vi "BaseProvider_ConfigurationMemory.vi"(1 "WireConfiguration":T2={"Edge thickness"=1, "Edge color"=5667411, "Center thickness"=1, "Center pattern"=enum."Solid", "CenterColor1"=9740924, "CenterColor2"=8694662, "Tunnels and terminals colors"=131187}, 2 "Icon":string="bluefull.png", 4 "Filter_Icons":bool, 5 "error in (no error)":errorcluster, 6 "Action":enum16{"Read", "Load", "Save", "Set"}(ring), 7 "PatternIn":T1 items=["4x4x4", "5x6x5", "6x8x6"]) -> (12 "ClassItemIconGroup":string[](array[string]), 13 "PatternOut":T1 items=["4x4x4", "5x6x5", "6x8x6"], 15 "WireConfigurationOut":T2={"Edge thickness"=1, "Edge color"=5667411, "Center thickness"=1, "Center pattern"=enum."Solid", "CenterColor1"=9740924, "CenterColor2"=8694662, "Tunnels and terminals colors"=131187}, 16 "IconOut":string="bluefull.png", 17 "ClassItemIconPaths":path[](array[path]), 18 "ClassItemIconNames":string[](array[string]), 19 "error out":errorcluster)   [LabVIEW 2020]
uses:
  SubVIs/GOOP_WireConfigurationType.ctl
  SubVIs/GOOP_WirePattern.ctl
  Common/ScriptingFunctions/Scripting_ConnectorPanePatternType.ctl
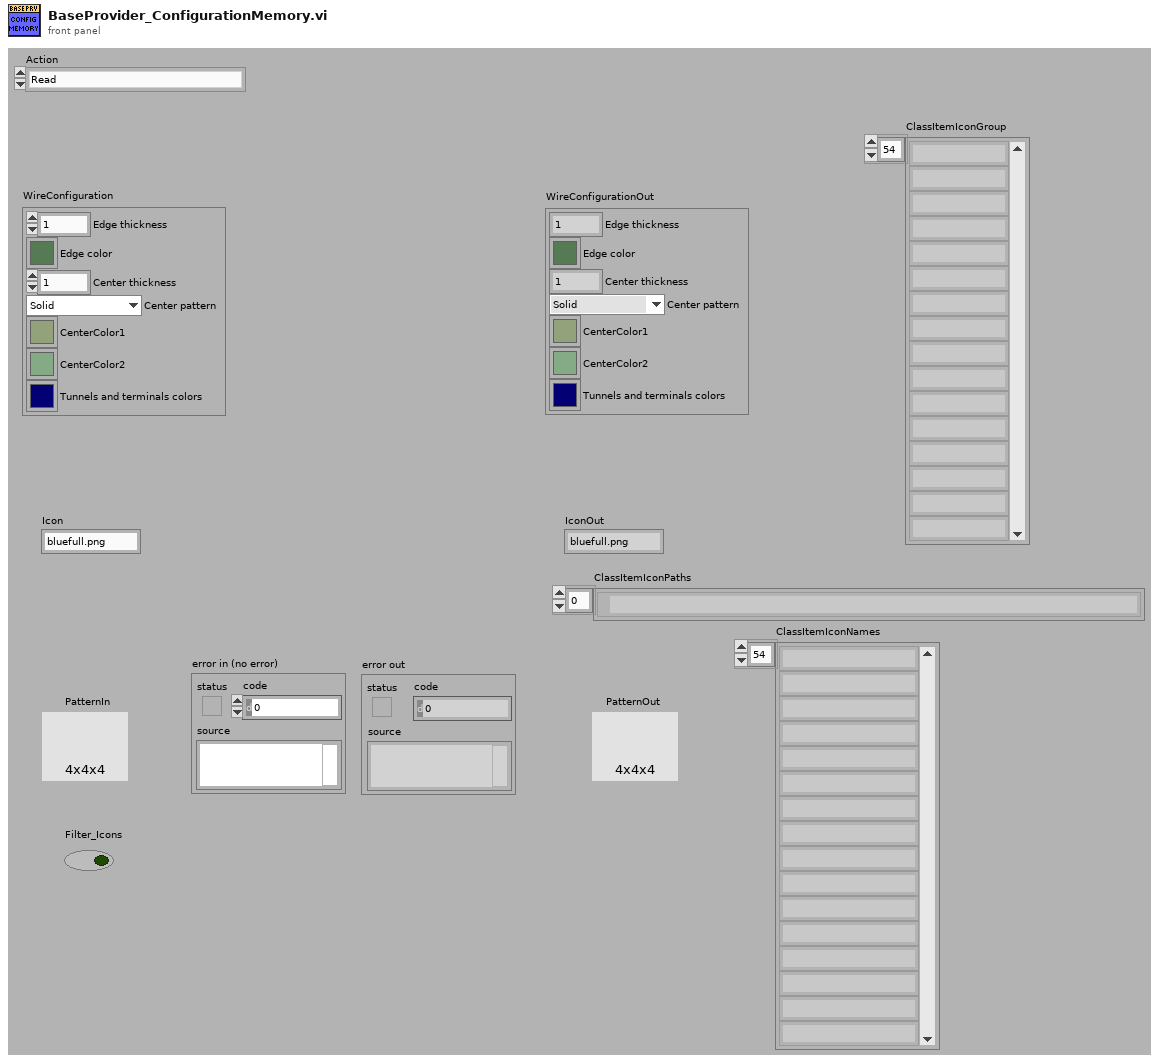
[diagram p1: front panel]
types:
  T1 = typedef "Scripting_ConnectorPanePatternType.ctl" = u16
  T2 = typedef "GOOP_WireConfigurationType.ctl" = cluster{"Edge thickness":i32, "Edge color":u32, "Center thickness":i32, "Center pattern":T3, "CenterColor1":u32, "CenterColor2":u32, "Tunnels and terminals colors":u32}
  T3 = typedef "GOOP_WirePattern.ctl" = enum16{"Solid", "Large dash", "Small dash"}
  T4 = cluster{"WireConfiguration":T2, "Icon":string, "Pattern":T1}
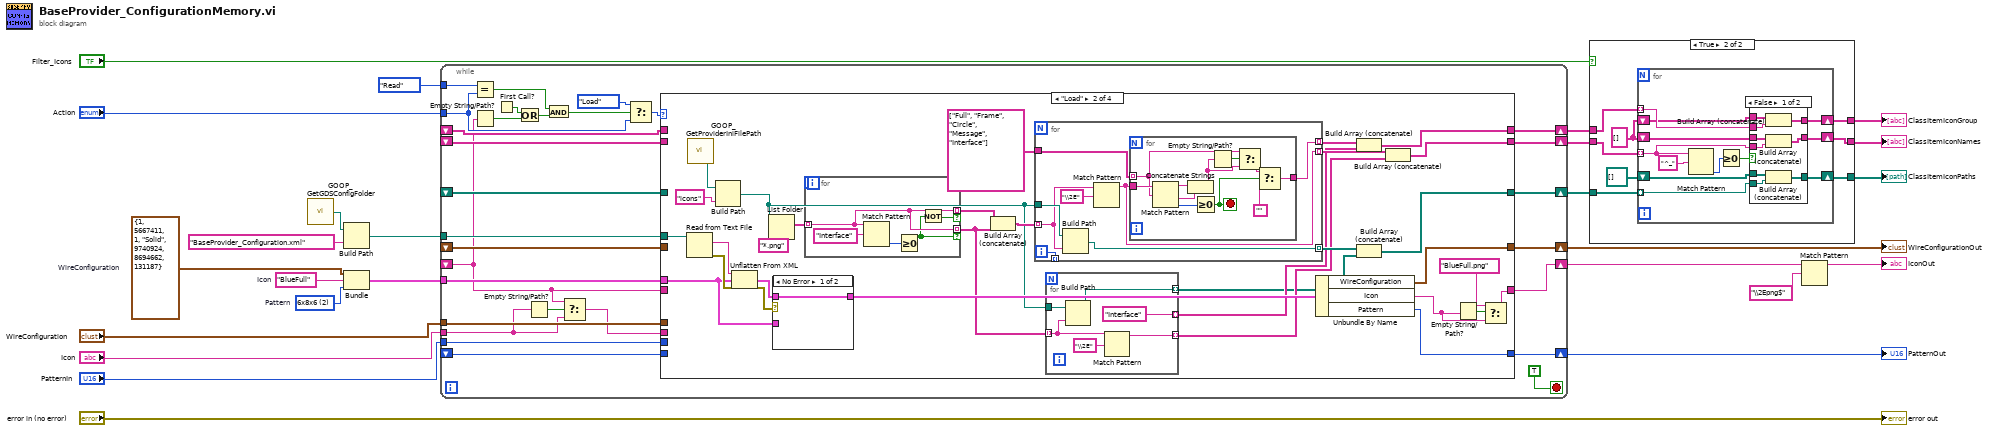
[diagram p0: block diagram]
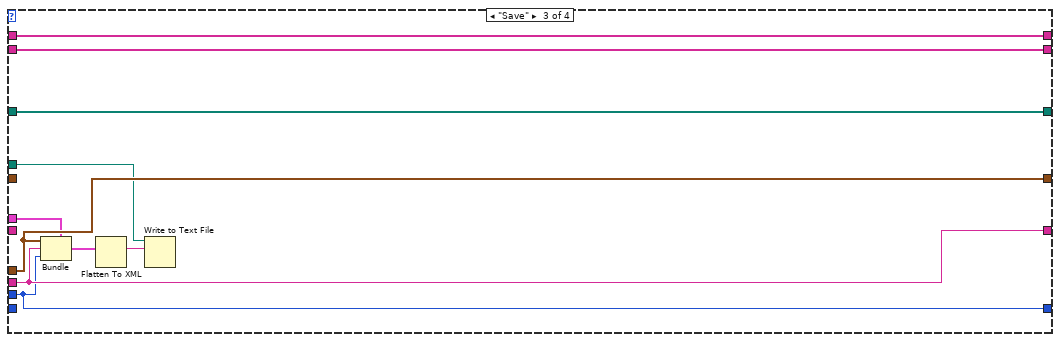
[diagram p6: hidden frame]
diagram:
  w15 = T1 2 items=["4x4x4", "5x6x5", "6x8x6"]  # Pattern
  w21 = "BlueFull"  # Icon
  w22 = T2 {"Edge thickness"=1, "Edge color"=5667411, "Center thickness"=1, "Center pattern"=enum."Solid", "CenterColor1"=9740924, "CenterColor2"=8694662, "Tunnels and terminals colors"=131187}  # WireConfiguration
  n1 = call "GOOP_GetGDSConfigFolder.vi"() -> ("GDSFolderPath"=w24:path)
  n2 = Build Path(base path=w24, name or relative path="BaseProvider_Configuration.xml") -> (appended path=w23:path)
  n3 = Bundle("WireConfiguration"=w22, "Icon"=w21, "Pattern"=w15) -> (w20:T4)  [unwired: 1 in]
  n4 = while {
    tunnel: "Action" -> [w32]
    tunnel: w23 -> [w54]
    tunnel: w20 -> [w53]
    shift-right: [w51] -> w19
    shift-left: _ -> [w49]
    shift-right: [w50] -> w2
    shift-left: _ -> [w28]
    shift-right: [w48] -> w11
    shift-left: _ -> [w47]
    shift-right: [w46] -> w12
    shift-left: _ -> [w45]
    tunnel: "WireConfiguration" -> [w44]
    tunnel: "Icon" -> [w26]
    shift-right: [w42] -> w13
    shift-left: _ -> [w41]
    tunnel: "PatternIn" -> [w43]
    shift-right: [w40] -> w10
    shift-left: _ -> [w39]
    tunnel: enum16{"Read", "Load", "Save", "Set"}."Read" ("t") -> [w38]
    stop <- TRUE stop-if-true
    n5 = Equal?(x=w38, y=w32) -> (x = y?=w34:bool)
    n6 = Empty String/Path?(string/path=w28) -> (empty?=w37:bool)
    n7 = First Call?() -> (First Call?: T/F=w36:bool)
    n8 = Or(x=w36, y=w37) -> (x .or. y?=w35:bool)
    n9 = Empty String/Path?(string/path=w26) -> (empty?=w29:bool)
    n10 = And(x=w34, y=w35) -> (x .and. y?=w33:bool)
    n11 = Select(t=w28, s=w29, f=w26) -> (s? t:f=w27:string)
    n12 = Select(t=enum16{"Read", "Load", "Save", "Set"}."Load", s=w33, f=w32) -> (s? t:f=w31:enum16{"Read", "Load", "Save", "Set"})
    n13 = case shown="\"Load\"" w31 {
      tunnel: w54 -> [_ w86 w124 _]
      tunnel: w53 -> [_ w85 w127 _]
      tunnel: [w60 w84 w129 w137] -> w51
      tunnel: [w59 w61 w128 w136] -> w50
      tunnel: w49 -> [w60 _ _ _]
      tunnel: w28 -> [w59 _ _ _]
      tunnel: [w58 w67 w133 w139] -> w48
      tunnel: w47 -> [w58 _ w133 w139]
      tunnel: [w57 w71 w131 w138] -> w46
      tunnel: w45 -> [w57 _ w131 w138]
      tunnel: w44 -> [_ _ w129 w137]
      tunnel: w27 -> [_ _ w128 w136]
      tunnel: w43 -> [_ _ w126 w135]
      tunnel: [w56 w80 w126 w135] -> w42
      tunnel: w41 -> [w56 _ _ _]
      tunnel: [w55 w72 w125 w134] -> w40
      tunnel: w39 -> [w55 _ w125 w134]
      frame "Read", Default {
      }
      frame "Load" {
        n14 = Read from Text File(file (use dialog)=w86) -> (text=w87:string, error out=w88:errorcluster)  [unwired: 3 in, 2 out]
        n15 = call "GOOP_GetProviderIniFilePath.vi"() -> ("ProviderMainFolder"=w81:path)  [unwired: 10 in, 1 out]
        n16 = Build Path(base path=w81, name or relative path="icons") -> (appended path=w66:path)
        n17 = Unflatten From XML(xml string=w87, type=w85, error in (no error)=w88) -> (value=w90:T4, error out=w89:errorcluster)
        n18 = List Folder(path=w66, pattern="*.png") -> (filenames=w75:string[])  [unwired: 2 in, 3 out]
        n19 = case shown="No Error" w89 {
          tunnel: w90 -> [w122 _]
          tunnel: [w122 w123] -> w91
          tunnel: w85 -> [_ w123]
          frame No Error {
          }
          frame Error {
          }
        }
        n20 = for {
          tunnel: w75 -> [w100] mode=indexing
          tunnel: [w100] -> w74 mode=indexing if=w99
          tunnel: [w100] -> w70 mode=indexing if=w98
          n21 = Match Pattern(string=w100, regular expression="Interface" ("name or relative path")) -> (offset past match=w101:i32)  [unwired: 1 in, 3 out]
          n22 = Greater Or Equal To 0?(x=w101) -> (x >= 0?=w98:bool)
          n23 = Not(x=w98) -> (.not. x?=w99:bool)
        }
        n24 = Build Array (concatenate)(w74, w70) -> (w73:string[])
        n25 = for {
          tunnel: w73 -> [w107] mode=indexing
          tunnel: w66 -> [w110]
          tunnel: string[] ["Full", "Frame", "Circle", "Message", "Interface"] -> [w108]
          tunnel: [w106] -> w78 mode=indexing
          tunnel: [w105] -> w77 mode=indexing
          tunnel: [w104] -> w76 mode=indexing
          tunnel: [w103] -> _ mode=indexing
          i -> [w103]
          n26 = Build Path(base path=w110, name or relative path=w107) -> (appended path=w106:path)
          n27 = Match Pattern(string=w107, regular expression="\\2E") -> (before substring=w105:string)  [unwired: 1 in, 3 out]
          n28 = for {
            tunnel: w105 -> [w121]
            tunnel: w108 -> [w113] mode=indexing
            tunnel: [w118] -> w104
            stop <- w119 stop-if-true
            n29 = Match Pattern(string=w121, regular expression=w113) -> (before substring=w116:string, after substring=w115:string, offset past match=w120:i32)  [unwired: 1 in, 1 out]
            n30 = Concatenate Strings(w116, w115) -> (w112:string)
            n31 = Greater Or Equal To 0?(x=w120) -> (x >= 0?=w119:bool)
            n32 = Empty String/Path?(string/path=w112) -> (empty?=w114:bool)
            n33 = Select(t=w113, s=w114, f=w112) -> (s? t:f=w111:string)
            n34 = Select(t=w111, s=w119, f="") -> (s? t:f=w118:string)
          }
        }
        n35 = for {
          tunnel: w70 -> [w94] mode=indexing
          tunnel: [w96] -> w69 mode=indexing
          tunnel: ["Interface" ("name or relative path")] -> w68 mode=indexing
          tunnel: w66 -> [w93]
          tunnel: [w92] -> w65 mode=indexing
          n36 = Build Path(base path=w93, name or relative path=w94) -> (appended path=w92:path)
          n37 = Match Pattern(string=w94, regular expression="\\2E") -> (before substring=w96:string)  [unwired: 1 in, 3 out]
        }
        n38 = Unbundle By Name(w91) -> ("WireConfiguration"=w84:T2, "Icon"=w62:string, "Pattern"=w80:T1)
        n39 = Build Array (concatenate)(w76, w68) -> (w72:string[])
        n40 = Build Array (concatenate)(w78, w65) -> (w67:path[])
        n41 = Build Array (concatenate)(w77, w69) -> (w71:string[])
        n42 = Empty String/Path?(string/path=w62) -> (empty?=w64:bool)
        n43 = Select(t="BlueFull.png" ("name or relative path"), s=w64, f=w62) -> (s? t:f=w61:string)
      }
      frame "Save" {
        n44 = Bundle(cluster=w127, "WireConfiguration"=w129, "Icon"=w128, "Pattern"=w126) -> (w130:T4)
        n45 = Flatten To XML(6:w130) -> (2:w132:string)
        n46 = Write to Text File(file (use dialog)=w124, text=w132) -> ()  [unwired: 2 in, 3 out]
      }
      frame "Set" {
      }
    }
  }
  "WireConfigurationOut" <- w19
  "PatternOut" <- w13
  n47 = case shown="True" "Filter_Icons" {
    tunnel: w12 -> [w141 w150]
    tunnel: w11 -> [w142 w149]
    tunnel: w10 -> [w140 w148]
    tunnel: [w142 w145] -> w9
    tunnel: [w141 w144] -> w8
    tunnel: [w140 w143] -> w7
    frame False {
    }
    frame True {
      w146 = string[] []
      n48 = for {
        tunnel: w150 -> [w157] mode=indexing
        tunnel: w149 -> [w159] mode=indexing
        tunnel: w148 -> [w158] mode=indexing
        shift-right: [w152] -> w145
        shift-left: path[] [] -> [w151]
        shift-right: [w153] -> w144
        shift-left: w146 -> [w154]
        shift-right: [w156] -> w143
        shift-left: w146 -> [w155]
        n49 = Match Pattern(string=w157, regular expression="^_") -> (offset past match=w161:i32)  [unwired: 1 in, 3 out]
        n50 = Greater Or Equal To 0?(x=w161) -> (x >= 0?=w160:bool)
        n51 = case shown="False" w160 {
          tunnel: w159 -> [w171 _]
          tunnel: w158 -> [w169 _]
          tunnel: w157 -> [w170 _]
          tunnel: [w168 w172] -> w156
          tunnel: w155 -> [w167 w172]
          tunnel: w154 -> [w166 w173]
          tunnel: [w165 w173] -> w153
          tunnel: [w164 w174] -> w152
          tunnel: w151 -> [w163 w174]
          frame False {
            n52 = Build Array (concatenate)(w167, w169) -> (w168:string[])
            n53 = Build Array (concatenate)(w166, w170) -> (w165:string[])
            n54 = Build Array (concatenate)(w163, w171) -> (w164:path[])
          }
          frame True {
          }
        }
      }
    }
  }
  "ClassItemIconPaths" <- w9
  "ClassItemIconNames" <- w8
  "ClassItemIconGroup" <- w7
  n55 = Match Pattern(string=w2, regular expression="\\2Epng$") -> (before substring=→"IconOut":string)  [unwired: 1 in, 3 out]
  "error out" <- "error in (no error)"
